vi "UI_Board_Geometry.vi"(11 "error in":errorcluster) -> (4 "Origin":i32=30, 6 "Cell":i32=38, 8 "Size":i32=592, 15 "error out":errorcluster)   [LabVIEW 2026]
doc: "바둑판 그리기와 좌표 변환이 같이 쓰는 상수. X = Origin + Col*Cell, Y = Origin + Row*Cell."
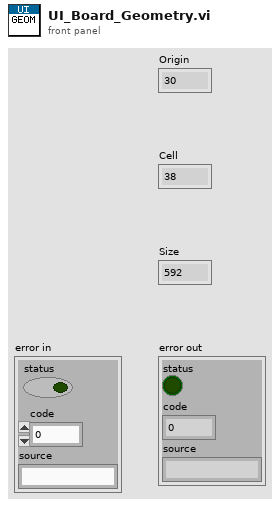
[diagram p1: front panel]
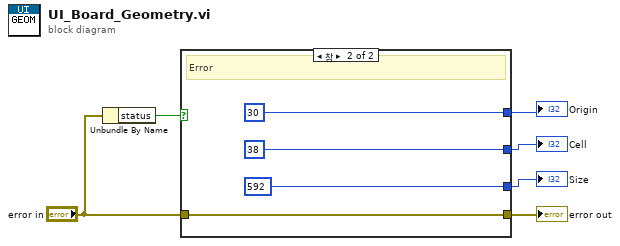
[diagram p0: block diagram]
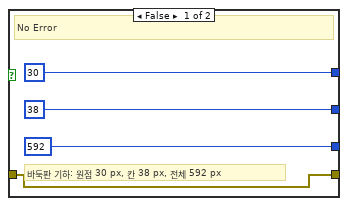
[diagram p2: hidden frame]
diagram:
  n1 = Unbundle By Name("error in") -> ("status"=w2:bool)
  n2 = case shown="참" w2 {
    tunnel: "error in" -> [w7 w11]
    tunnel: [30 30] -> w3
    tunnel: [38 38] -> w4
    tunnel: [592 592] -> w5
    tunnel: [w7 w11] -> w6
    frame False {
      # "바둑판 기하: 원점 30 px, 칸 38 px, 전체 592 px"
      # "No Error"
    }
    frame True {
      # "Error"
    }
  }
  "Origin" <- w3
  "Cell" <- w4
  "Size" <- w5
  "error out" <- w6
